vi "Complete Request.vi"(7 "Processing In":refnum<class "Processing.lvclass">, 11 "WebSocket Handler in":refnum<class "WebSocket Handler.lvclass">) -> (0 "error out":errorcluster, 5 "Processing":refnum<class "Processing.lvclass">)   [LabVIEW 2020, in "HTTP Server.lvlib" / "WebSocket Handler.lvclass"]
uses:
  WebSocket Handler.lvclass
  Processing/Processing.lvclass
  Processing/Processing.lvclass/Processing.ctl
  WebSocket Client/WebSocket Client.lvclass
  lv-http-util/HTTP Utils/Request/Request.lvclass/Request.ctl
  lv-http-util/HTTP Utils/Request/Request.lvclass
  lv-uri/URI/URI/URI.lvclass
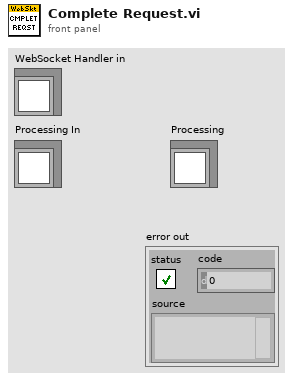
[diagram p1: front panel]
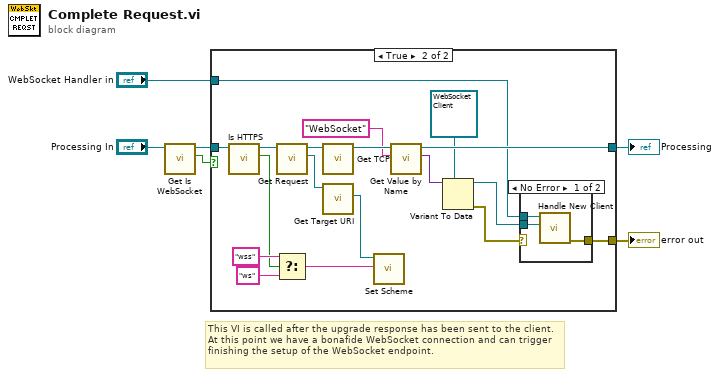
[diagram p0: block diagram]
diagram:
  # "This VI is called after the upgrade response has been sent to the client. At this point we have a bonafide WebSocket connection and can trigger finishing the setup of the WebSocket endpoint."
  n1 = call "Get Is WebSocket.vi"("Processing in"="Processing In") -> ("Is WebSocket"=w6:bool, "Processing out"=w5:refnum<class "Processing.lvclass">)  [unwired: 9 in]
  n2 = case shown="True" w6 {
    tunnel: w5 -> [w7 w23]
    tunnel: [w7 w15] -> w3
    tunnel: "WebSocket Handler in" -> [_ w9]
    tunnel: [_ w18] -> w1
    frame False {
    }
    frame True {
      n3 = call "Is HTTPS.vi"("Processing in"=w23) -> ("HTTPS?"=w20:bool, "Processing out"=w17:refnum<class "Processing.lvclass">)  [unwired: 8 in, 1 out]
      n4 = call "Get Request.vi"("Processing in"=w17) -> ("Request"=w14:refnum<class "Request.lvclass">, "Processing out"=w16:refnum<class "Processing.lvclass">)  [unwired: 9 in]
      n5 = Select(t="wss", s=w20, f="ws") -> (s? t:f=w19:string)
      n6 = call "Get TCP.vi"("Processing in"=w16) -> ("Processing out"=w24:refnum<class "Processing.lvclass">)  [unwired: 9 in, 1 out]
      n7 = call "Get Target URI.vi"("Request in"=w14) -> ("Target URI"=w10:refnum<class "URI.lvclass">)  [unwired: 8 in, 2 out]
      n8 = call "Set Scheme.vi"("Scheme"=w19, "URI in"=w10) -> ()  [unwired: 9 in, 1 out]
      n9 = call "Get Value by Name.vi"("Name"="WebSocket" ("Name for Type"), "Processing in"=w24) -> ("Value"=w13:variant, "Processing out"=w15:refnum<class "Processing.lvclass">)  [unwired: 7 in, 1 out]
      n10 = Variant To Data(type=refnum<class "WebSocket Client.lvclass"> refnum ("WebSocket"), Variant=w13) -> (data=w8:refnum<class "WebSocket Client.lvclass">, error out=w25:errorcluster)  [unwired: 1 in]
      n11 = case shown="No Error" w25 {
        selector: w25 -> [_ w29]
        tunnel: [w27 w29] -> w18
        tunnel: w9 -> [w28 _]
        tunnel: w8 -> [w26 _]
        frame No Error {
          n12 = call "Handle New Client.vi"("WS Client"=w26, "WebSocket Handler in"=w28) -> ("error out"=w27:errorcluster)  [unwired: 8 in, 1 out]
        }
        frame Error {
        }
      }
    }
  }
  "error out" <- w1
  "Processing" <- w3
